vi "B_region_selection for ANAL.vi"(8 "datapoint":i64=10000, 9 "B_END [s]":dbl format="%#_13g", 10 "B_Start [s]":dbl format="%#_13g", 11 "Raw data":dbl[](array[numeric])) -> (0 "Selected Raw D":T1, 2 "Selected Time":dbl[](array[numeric]), 3 "Selected Raw data":dbl[](array[numeric]))   [LabVIEW 2018]
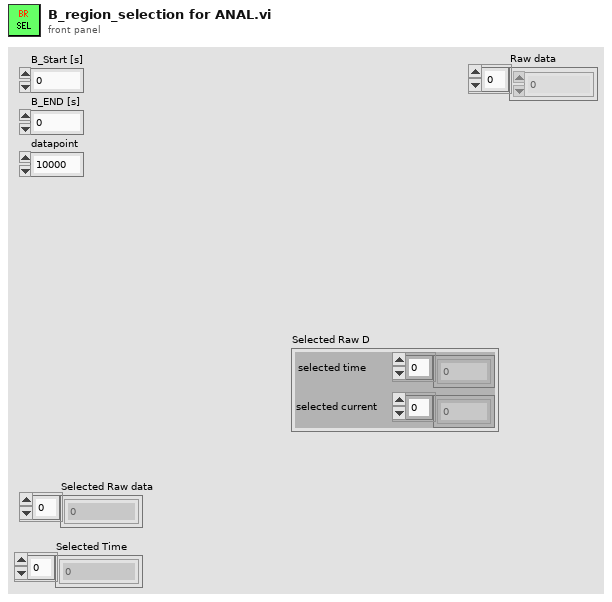
[diagram p1: front panel]
types:
  T1 = cluster{"selected time":dbl[], "selected current":dbl[]}
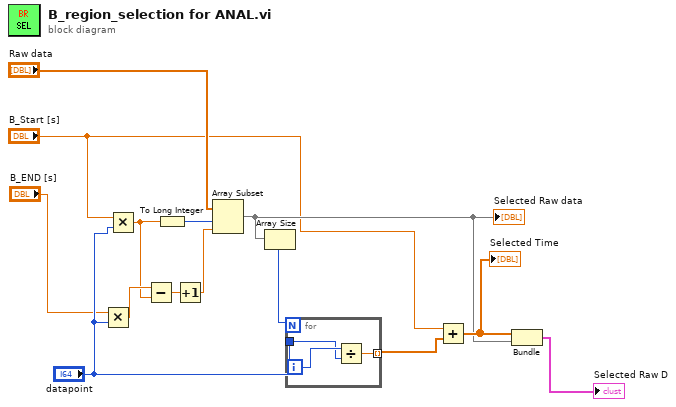
[diagram p0: block diagram]
diagram:
  n1 = Multiply(x="B_END [s]", y="datapoint") -> (x*y=w14:dbl)
  n2 = Multiply(x="B_Start [s]", y="datapoint") -> (x*y=w13:dbl)
  n3 = Subtract(x=w14, y=w13) -> (x-y=w8:dbl)
  n4 = To Long Integer(number=w13) -> (32bit integer=w12:i32)
  n5 = Increment(x=w8) -> (x+1=w7:dbl)
  n6 = Array Subset(array="Raw data", index=w12, length=w7) -> (w5:dbl[])
  "Selected Raw data" <- w5
  n7 = Array Size(array=w5) -> (size(s)=w11:i32)
  n8 = for {
    N: w11 -> [_]
    tunnel: "datapoint" -> [w16]
    tunnel: [w15] -> w9 mode=indexing
    i -> [w17]
    n9 = Divide(x=w17, y=w16) -> (x/y=w15:dbl)
  }
  n10 = Add(x="B_Start [s]", y=w9) -> (x+y=w6:dbl[])
  "Selected Time" <- w6
  n11 = Bundle(w6, w5) -> (→"Selected Raw D":cluster{dbl[], dbl[]})  [unwired: 1 in]
